vi "Handle OpModes.vi"(11 "OpModes":T1) -> ()   [LabVIEW 2023]
doc: "As directed by the driver station protocol, start opModes and if needed, abort them."
uses:
  <vilib>/MRC/MrcLib.lvlib
  FRC_NetworkTablesLV.so
  <vilib>/MRC/MrcLib/VIs/Robot Framework/DS OpModes.ctl
panel:
  out "timed out":bool
  out "OpMode History":string
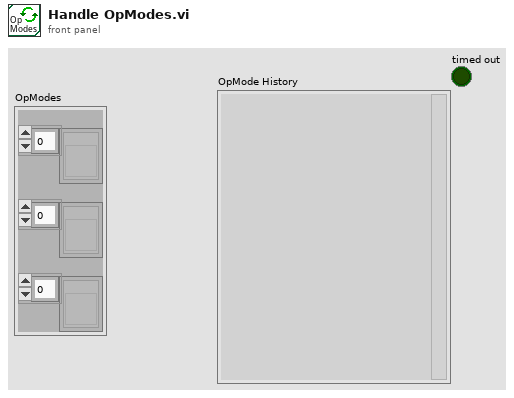
[diagram p1: front panel]
types:
  T1 = typedef "DS OpModes.ctl" = cluster{"Autos":refnum<vi>[], "Teles":refnum<vi>[], "Utilities":refnum<vi>[]}
  T2 = enum32{"Bad", "Idle", "Run top level", "Running"}
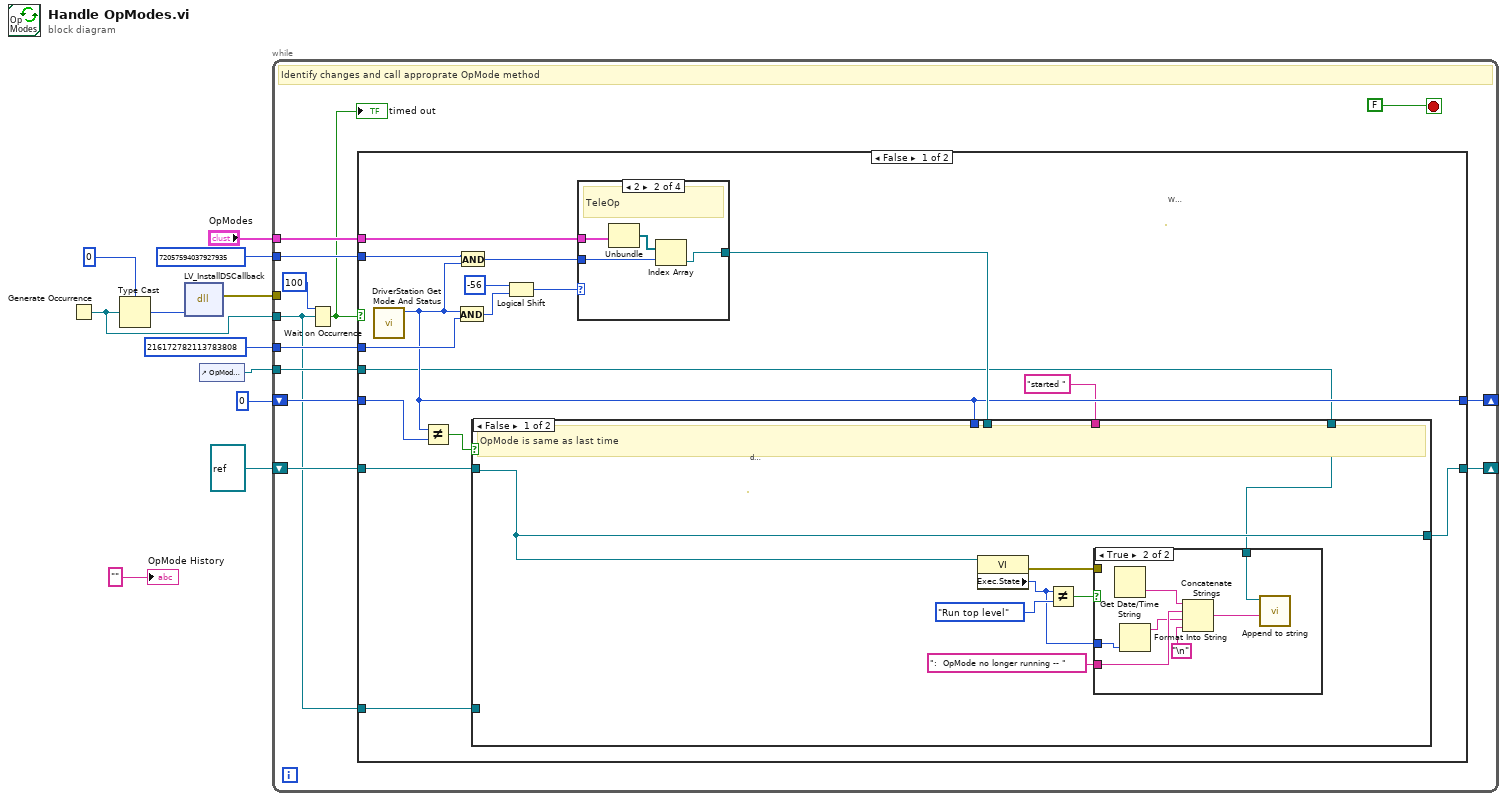
[diagram p0: block diagram]
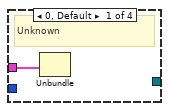
[diagram p2: hidden frame]
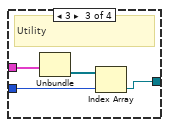
[diagram p3: hidden frame]
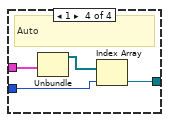
[diagram p4: hidden frame]
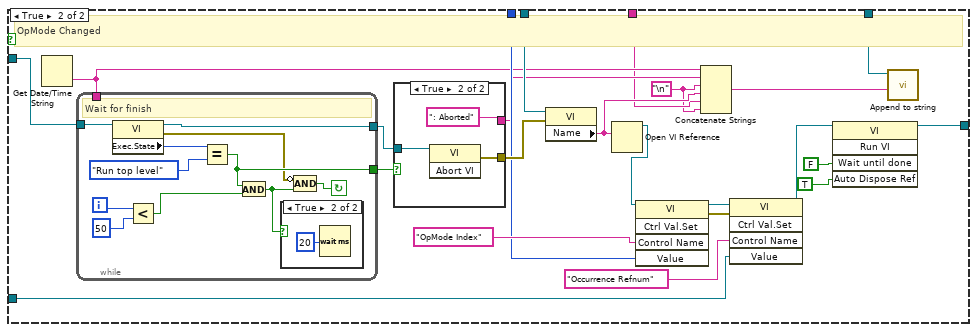
[diagram p6: hidden frame]
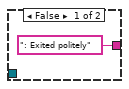
[diagram p7: hidden frame]
diagram:
  n1 = Generate Occurrence() -> (w1:refnum<k4>)
  n2 = Type Cast(type=u32 0, x=w1) -> (*(type *) &x=w4:u32)
  n3 = dll-call lib="FRC_NetworkTablesLV.*" fn="LV_InstallDSCallback"("occurrence"=w4) -> (error out=w2:errorcluster)  [unwired: 5 in, 1 out]
  n4 = control-ref of="OpMode History"() -> (w5:refnum<vi>)
  n5 = while {
    tunnel: "OpModes" -> [w21]
    tunnel: u64 216172782113783808 ("y") -> [w22]
    tunnel: u64 72057594037927935 ("y") -> [w20]
    shift-right: [w16] -> _
    shift-left: u8 0 ("RobotMode") -> [w19]
    shift-right: [w17] -> _
    shift-left: refnum<vi> refnum ("vi reference") -> [w18]
    tunnel: w5 -> [w15]
    tunnel: w2 -> [_]
    tunnel: w1 -> [w12]
    stop <- FALSE stop-if-true
    # "Identify changes and call approprate OpMode method"
    n6 = Wait on Occurrence(2:w12, 3:100 ("ms timeout (-1)")) -> (0:w13:bool)  [unwired: 1 in]
    "timed out" <- w13
    n7 = case shown="False" w13 {
      tunnel: w22 -> [w39 _]
      tunnel: w21 -> [w36 _]
      tunnel: w20 -> [w35 _]
      tunnel: w19 -> [w33 w107]
      tunnel: w18 -> [w30 w106]
      tunnel: [w29 w106] -> w17
      tunnel: [w27 w107] -> w16
      tunnel: w15 -> [w25 _]
      tunnel: w12 -> [w24 _]
      frame False {
        # "Write a better\ntrace string ???"
        n8 = call <vilib>:"DriverStation Get Mode And Status.vi"() -> ("currentOpMode"=w27:u64)  [unwired: 6 in, 5 out]
        n9 = Not Equal?(x=w27, y=w33) -> (x != y?=w32:bool)
        n10 = And(x=w27, y=w39) -> (x .and. y?=w38:u64)
        n11 = And(x=w35, y=w27) -> (x .and. y?=w28:u64)
        n12 = Logical Shift(y=i16 -56, x=w38) -> (x << y=w34:u64)
        n13 = case shown="2" w34 {
          tunnel: w36 -> [w40 w44 w48 w52]
          tunnel: w28 -> [_ w42 w45 w50]
          tunnel: [_ w41 w46 w49] -> w31
          frame 0, Default {
            # "Unknown"
            n14 = Unbundle(w40) -> ()  [unwired: 3 out]
          }
          frame 2 {
            # "TeleOp"
            n15 = Unbundle(w44) -> ("Teles"=w43:refnum<vi>[])  [unwired: 2 out]
            n16 = Index Array(array=w43, index=w42) -> (element=w41:refnum<vi>)
          }
          frame 3 {
            # "Utility"
            n17 = Unbundle(w48) -> ("Utilities"=w47:refnum<vi>[])  [unwired: 2 out]
            n18 = Index Array(array=w47, index=w45) -> (element=w46:refnum<vi>)
          }
          frame 1 {
            # "Auto"
            n19 = Unbundle(w52) -> ("Autos"=w51:refnum<vi>[])  [unwired: 2 out]
            n20 = Index Array(array=w51, index=w50) -> (element=w49:refnum<vi>)
          }
        }
        n21 = case shown="False" w32 {
          tunnel: w31 -> [_ w87]
          tunnel: w30 -> [w59 w85]
          tunnel: [w59 w86] -> w29
          tunnel: w27 -> [_ w79]
          tunnel: "started " -> [_ w75]
          tunnel: w25 -> [w54 w72]
          tunnel: w24 -> [_ w67]
          frame False {
            # "delay ???"
            # "OpMode is same as last time"
            n22 = property class="VI"(reference=w59) -> (error out=w53:errorcluster, "Exec.State"=w55:T2)  [unwired: 1 in, 1 out]
            n23 = Not Equal?(x=w55, y=T2."Run top level" ("Execution:State")) -> (x != y?=w57:bool)
            n24 = case shown="True" w57 {
              tunnel: ":  OpMode no longer running -- " -> [_ w65]
              tunnel: w55 -> [_ w64]
              tunnel: w54 -> [_ w60]
              tunnel: w53 -> [_ _]
              frame False {
              }
              frame True {
                n25 = Get Date/Time String() -> (time string=w66:string)  [unwired: 3 in, 1 out]
                n26 = Format Into String(w64) -> (resulting string=w63:string)  [unwired: 3 in, 1 out]
                n27 = Concatenate Strings(w66, w65, w63, "\n") -> (w61:string)
                n28 = call <vilib>:"Append to string.vi"("string"=w61, "Str Refnum"=w60) -> ()  [unwired: 10 in]
              }
            }
          }
          frame True {
            w74 = "\n"
            # "OpMode Changed"
            n29 = Get Date/Time String() -> (time string=w78:string)  [unwired: 3 in, 1 out]
            n30 = while {
              tunnel: w85 -> [w104]
              tunnel: [w98] -> w84
              tunnel: [w97] -> w83
              tunnel: w78 -> [_]
              i -> [w101]
              stop <- w95 continue-if-true
              # "Wait for finish"
              n31 = property class="VI"(reference=w104) -> (reference out=w98:refnum<vi>, error out=w94:errorcluster, "Exec.State"=w103:T2)  [unwired: 1 in]
              n32 = Less?(x=w101, y=50 ("x")) -> (x < y?=w99:bool)
              n33 = Equal?(x=w103, y=T2."Run top level" ("Execution:State")) -> (x = y?=w97:bool)
              n34 = And(x=w97, y=w99) -> (x .and. y?=w96:bool)
              n35 = case shown="True" w96 {
                frame False {
                }
                frame True {
                  n36 = Wait (ms)(milliseconds to wait=u32 20) -> ()  [unwired: 1 out]
                }
              }
              n37 = Compound Arithmetic op=AND(invert w94, w96) -> (w95:bool)
            }
            n38 = case shown="True" w83 {
              tunnel: w84 -> [_ w93]
              tunnel: [_ w92] -> w82
              tunnel: [": Exited politely" ("Control Name") ": Aborted" ("Control Name")] -> w77
              frame False {
              }
              frame True {
                n39 = invoke class="VI" method="Abort VI"(reference=w93) -> (error out=w92:errorcluster)  [unwired: 2 in, 2 out]
              }
            }
            n40 = property class="VI"(reference=w87, error in=w82) -> ("Name"=w76:string)  [unwired: 2 out]
            n41 = Open VI Reference(vi path=w76) -> (vi reference=w81:refnum<vi>)  [unwired: 5 in, 1 out]
            n42 = invoke class="VI" method="Ctrl Val.Set"(reference=w81, "Control Name"="OpMode Index", "Value"=w79) -> (reference out=w71:refnum<vi>, error out=w70:errorcluster)  [unwired: 2 in, 3 out]
            n43 = Concatenate Strings(w78, w77, w74, w76, w75, w74) -> (w73:string)
            n44 = invoke class="VI" method="Ctrl Val.Set"(reference=w71, error in=w70, "Control Name"="Occurrence Refnum", "Value"=w67) -> (reference out=w69:refnum<vi>)  [unwired: 1 in, 4 out]
            n45 = invoke class="VI" method="Run VI"(reference=w69, "Wait until done"=FALSE ("Wait Until Done"), "Auto Dispose Ref"=TRUE ("Auto Dispose Reference")) -> (reference out=w86:refnum<vi>)  [unwired: 2 in, 4 out]
            n46 = call <vilib>:"Append to string.vi"("string"=w73, "Str Refnum"=w72) -> ()  [unwired: 10 in]
          }
        }
      }
      frame True {
      }
    }
  }
  "OpMode History" <- "" ("OpMode History")
